vi "request SCPI Command.vi"(8 "error in (no error)":errorcluster, 10 "SCPI Command":string, 11 "LTE in":refnum<class "LTE.lvclass">) -> (0 "error out":errorcluster, 3 "LTE out":refnum<class "LTE.lvclass">)   [LabVIEW 2023, in "ANRITSU Call Box.lvlib" / "LTE.lvclass"]
uses:
  LTE.lvclass
  Type Definition/Call Device - Protocol Type Selector.ctl
  LTE.lvclass/LTE.ctl
  ANRITSU Call Box.lvlib
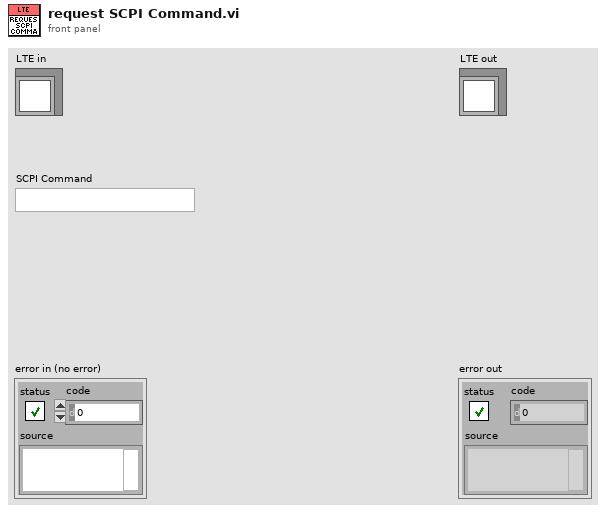
[diagram p1: front panel]
types:
  T1 = typedef "ANRITSU Call Box.lvlib/Call Device - Protocol Type Selector.ctl" = enum16{"8000A - NR", "8000A - LTE", "882xC - LTE"}
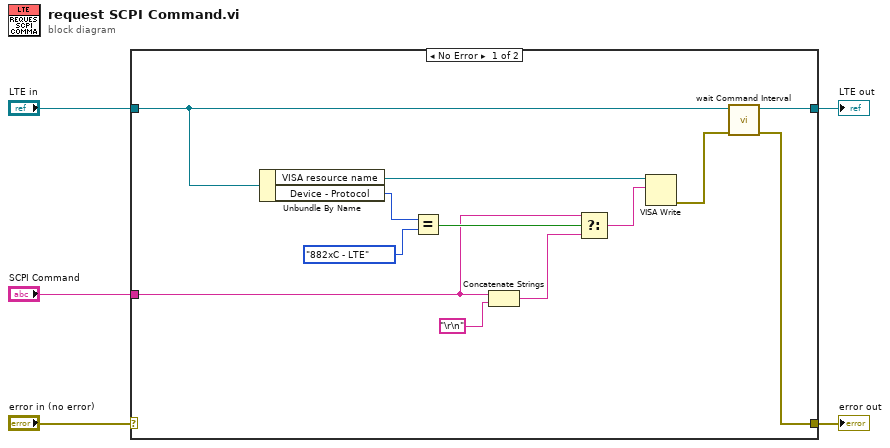
[diagram p0: block diagram]
diagram:
  n1 = case shown="No Error" "error in (no error)" {
    selector: "error in (no error)" -> [_ w19]
    tunnel: [w8 w19] -> w4
    tunnel: [w10 w18] -> w2
    tunnel: "LTE in" -> [w11 w18]
    tunnel: "SCPI Command" -> [w14 _]
    frame No Error {
      n2 = Unbundle By Name(w11) -> ("VISA resource name"=w6:refnum<visa-resource-name>, "Device - Protocol"=w7:T1)
      n3 = Equal?(x=w7, y=Call_Device_-_Protocol_Type_Selector."882xC - LTE") -> (x = y?=w15:bool)
      n4 = Concatenate Strings(w14, "\r\n") -> (w13:string)
      n5 = Select(t=w14, s=w15, f=w13) -> (s? t:f=w12:string)
      n6 = VISA Write(VISA resource name=w6, write buffer=w12) -> (error out=w9:errorcluster)  [unwired: 1 in, 2 out]
      n7 = call "wait Command Interval.vi"("error in (no error)"=w9, "LTE in"=w11) -> ("error out"=w8:errorcluster, "LTE out"=w10:refnum<class "LTE.lvclass">)  [unwired: 8 in]
    }
    frame Error {
    }
  }
  "error out" <- w4
  "LTE out" <- w2
